vi "I2C.vi"() -> ()   [LabVIEW 2012]
uses:
  USB2UARTSPIIICDLL.dll
panel:
  out "CloseUsb函数返回值":dbl
  in  "数组":i8[](array[numeric]) format="%x"
  out "IICSendData函数返回值":dbl
  out "ConfigIICParam函数返回值":dbl
  in  "IIC速率":dbl
  in  "开始测试按钮":bool
  out "OpenUsb函数返回值":dbl
  in  "UsbIndex":dbl
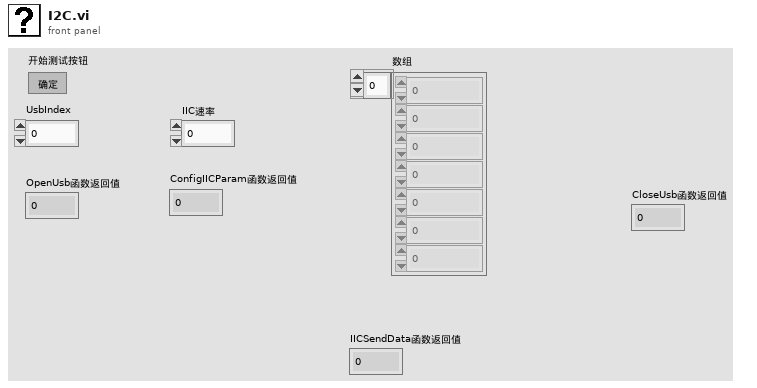
[diagram p1: front panel]
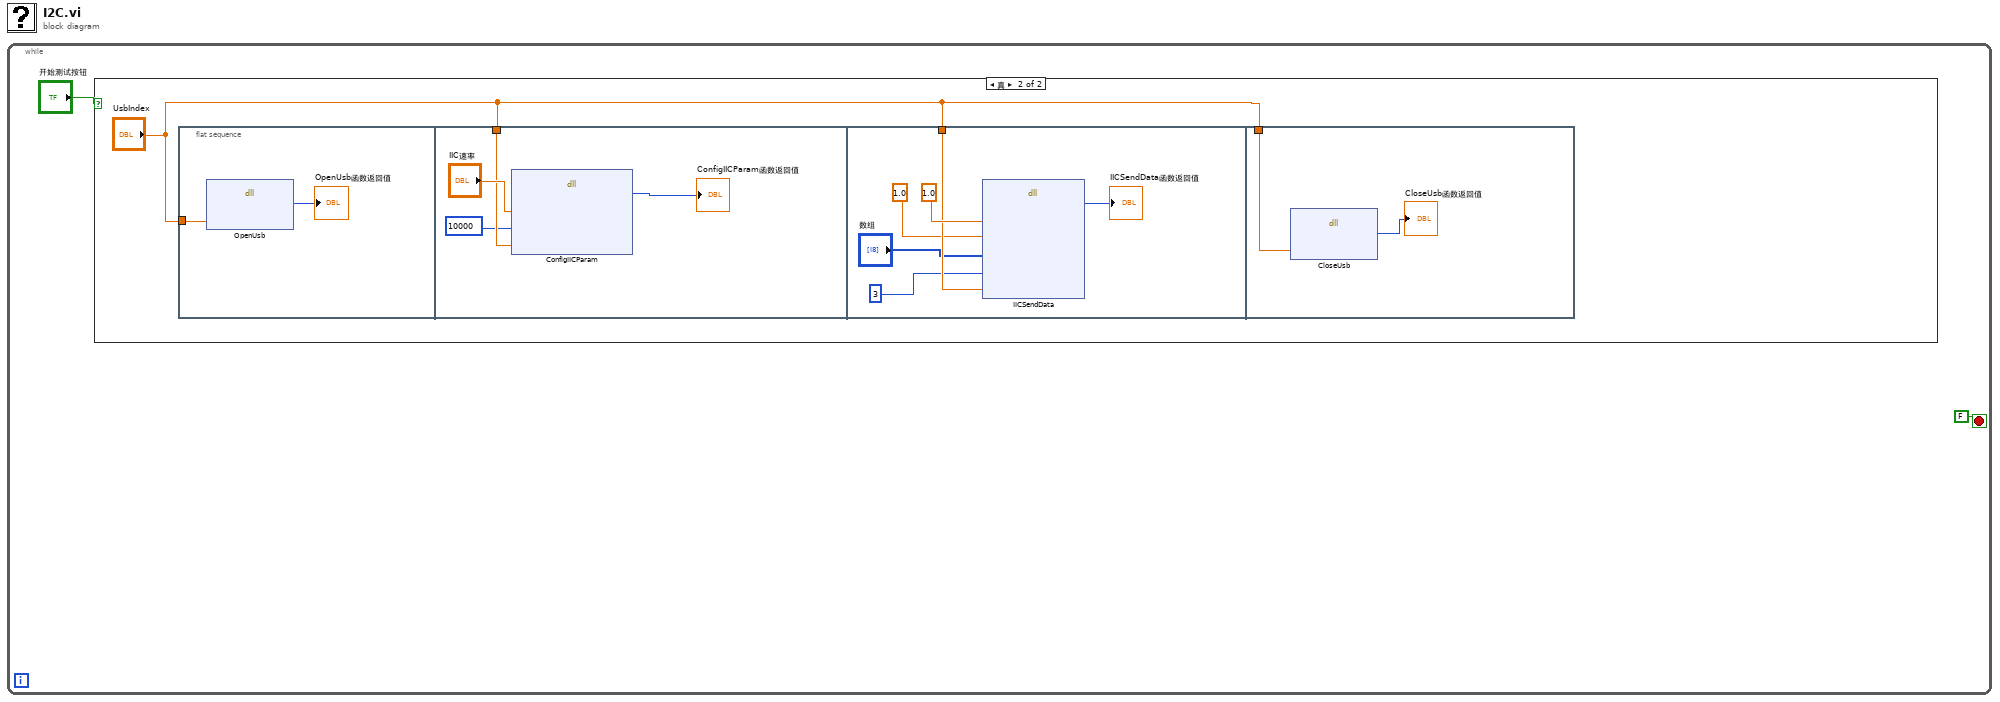
[diagram p0: block diagram]
diagram:
  n1 = while {
    stop <- FALSE stop-if-true
    n2 = case shown="真" "开始测试按钮" {
      frame False {
      }
      frame True {
        n3 = flat-sequence "平铺式顺序结构" {
          tunnel: "UsbIndex" -> [w5]
          tunnel: "UsbIndex" -> [w8]
          tunnel: "UsbIndex" -> [w13]
          tunnel: "UsbIndex" -> [w17]
          frame #0 {
            n4 = dll-call lib="F:/work/USB2SPIUARTIIC/103/SW/Labview/I2C/USB2UARTSPIIICDLL.dll" fn="OpenUsb"("UsbIndex"=w5) -> ("返回类型"=→"OpenUsb函数返回值":i32)  [unwired: 4 in, 2 out]
          }
          frame #1 {
            n5 = dll-call lib="F:/work/USB2SPIUARTIIC/103/SW/Labview/I2C/USB2UARTSPIIICDLL.dll" fn="ConfigIICParam"("rate"="IIC速率", "clkSLevel"=10000, "UsbIndex"=w8) -> ("返回类型"=→"ConfigIICParam函数返回值":i32)  [unwired: 6 in, 2 out]
          }
          frame #2 {
            n6 = dll-call lib="F:/work/USB2SPIUARTIIC/103/SW/Labview/I2C/USB2UARTSPIIICDLL.dll" fn="IICSendData"("strartBit"=1.0, "stopBit"=1.0 ("strartBit"), "sendBuf"="数组", "len"=i16 3 ("strartBit"), "UsbIndex"=w13) -> ("返回类型"=→"IICSendData函数返回值":i32)  [unwired: 8 in, 2 out]
          }
          frame #3 {
            n7 = dll-call lib="F:/work/USB2SPIUARTIIC/103/SW/Labview/I2C/USB2UARTSPIIICDLL.dll" fn="CloseUsb"("UsbIndex"=w17) -> ("返回类型"=→"CloseUsb函数返回值":i32)  [unwired: 4 in, 2 out]
          }
        }
      }
    }
  }
